vi "NestedMember.vi"(8 "error in":errorcluster) -> (0 "error out":errorcluster)   [LabVIEW 2024, in "NestedOwner.lvlib"]
doc: "A minimal owning-library path fixture. It forwards the required error cluster unchanged and has no other behavior."
uses:
  NestedOwner.lvlib
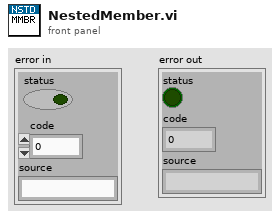
[diagram p1: front panel]
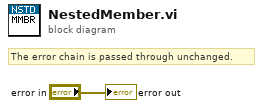
[diagram p0: block diagram]
diagram:
  # "The error chain is passed through unchanged."
  "error out" <- "error in"
